vi "Destroy.vi"(8 "error in (no error)":errorcluster, 11 "CIFTag in":refnum<class "CIF_CIPC_Chn.lvclass">) -> (0 "error out":errorcluster, 3 "CIFTag out":refnum<class "CIF_CIPC_Chn.lvclass">)   [LabVIEW 2021, in "CIF_CIPC_Chn.lvclass"]
uses:
  CIF_CIPC_Chn.lvclass
  C:/Program Files/National Instruments/LabVIEW 2021/vi.lib/CIF Foundation/CIF Channels Core/CIFChannels/CIFChannels.lvclass
  <vilib>/CIF Foundation/CIF Channels Core/ChannelCommon/typedef/Channel State.ctl
  Typedef/Buffer Configuration Data.ctl
  <vilib>/CIF Foundation/CIF CIPC/TypeDefs/Backpressure References.ctl
  <vilib>/CIF Foundation/CIF CIPC/TypeDefs/Backpressure Names.ctl
  <vilib>/CIF Foundation/CIF Channels Core/CIFChannels/CIFChannels.lvclass/CIFChannels.ctl
  CIF_CIPC_Chn.lvclass/CIF_CIPC_Chn.ctl
  <vilib>/CIF Foundation/CIF Channels Core/CIFChannels/Accessors/Read Direction.vi
  <vilib>/CIF Foundation/CIF Channels Core/CIFChannels/Accessors/Read FIFO Backpressure.vi
  Accessors/Read Buffer Configuration.vi
  Accessors/Read CIPC Channel.vi
  Accessors/Write Buffer Configuration.vi
  Accessors/Write CIPC Channel.vi
  <vilib>/CIF Foundation/CIF Channels Core/CIFChannels/Accessors/Write Subscriber Count.vi
  <vilib>/CIF Foundation/CIF Channels Core/CIFChannels/Accessors/Write Channel State.vi
  <vilib>/CIF Foundation/CIF CIPC/CIF_NI_CIPC.lvlib
  <vilib>/CIF Foundation/CIF Channels Core/ChannelCommon/ChannelCommon.lvlib
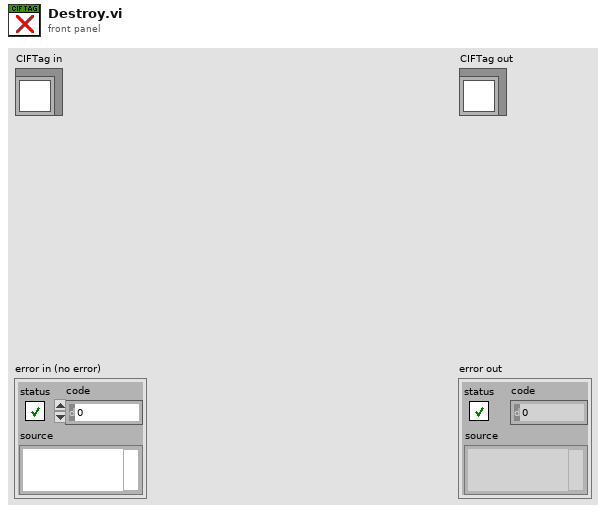
[diagram p1: front panel]
types:
  T1 = typedef "ChannelCommon.lvlib/Channel State.ctl" = enum8{"Creating", "Disconnected", "Connecting", "Connected", "Destroyed"}
  T2 = typedef "CIF_CIPC_Chn.lvclass/Buffer Configuration Data.ctl" = cluster{"Total Size":u32, "Read Size":u32, "Read Offset":u32, "CIPC BP References":T3, "CIPC Backpressure Names":T4, "Override CIPC Name":string, "Encoder Data":string}
  T3 = typedef "CIF_NI_CIPC.lvlib/Backpressure References.ctl" = cluster{"CIPC Reference":u64, "CIPC BP Reference":u64}
  T4 = typedef "CIF_NI_CIPC.lvlib/Backpressure Names.ctl" = cluster{"CIPC Name":string, "CIPC BP Name":string}
  T5 = typedef "ChannelCommon.lvlib/Direction.ctl" = enum8{"Publisher", "Subscriber"}
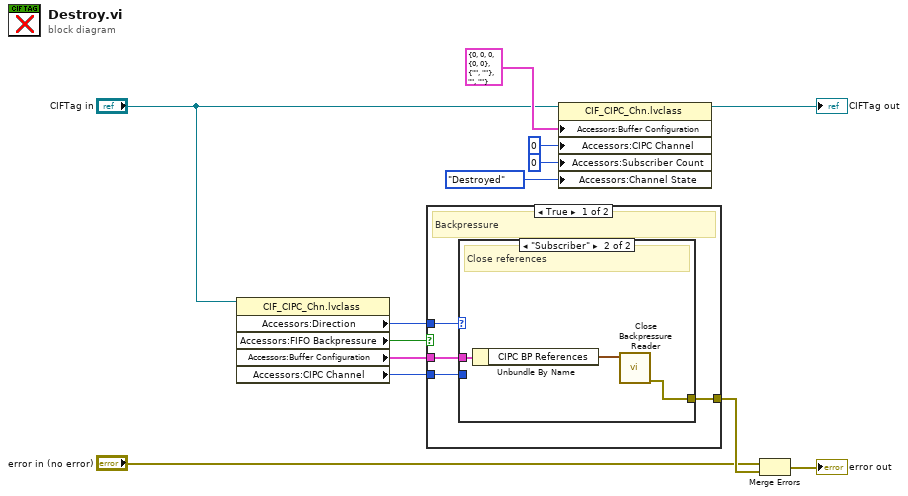
[diagram p0: block diagram]
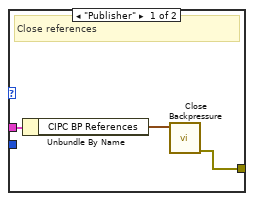
[diagram p2: hidden frame]
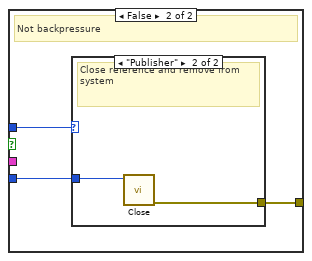
[diagram p3: hidden frame]
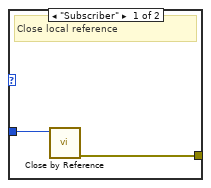
[diagram p4: hidden frame]
diagram:
  n1 = property class="CIF_CIPC_Chn.lvclass"(reference="CIFTag in") -> ("Accessors:Direction"=w13:T5, "Accessors:FIFO Backpressure"=w11:bool, "Accessors:Buffer Configuration"=w10:T2, "Accessors:CIPC Channel"=w12:u64)  [unwired: 1 in, 2 out]
  n2 = case shown="True" w11 {
    tunnel: w13 -> [w17 w26]
    tunnel: w12 -> [w16 w25]
    tunnel: [w14 w24] -> w9
    tunnel: w10 -> [w15 _]
    frame True {
      # "Backpressure"
      n3 = case shown="\"Subscriber\"" w17 {
        tunnel: w16 -> [_ _]
        tunnel: w15 -> [w20 w23]
        tunnel: [w18 w21] -> w14
        frame "Publisher" {
          # "Close references"
          n4 = Unbundle By Name(w20) -> ("CIPC BP References"=w19:T3)
          n5 = call <vilib>:"Close Backpressure.vi"("CIPC BP References in"=w19) -> ("error out"=w18:errorcluster)  [unwired: 10 in]
        }
        frame "Subscriber" {
          # "Close references"
          n6 = Unbundle By Name(w23) -> ("CIPC BP References"=w22:T3)
          n7 = call <vilib>:"Close Backpressure Reader.vi"("CIPC BP References in"=w22) -> ("error out"=w21:errorcluster)  [unwired: 10 in]
        }
      }
    }
    frame False {
      # "Not backpressure"
      n8 = case shown="\"Publisher\"" w26 {
        tunnel: w25 -> [w28 w30]
        tunnel: [w27 w29] -> w24
        frame "Subscriber" {
          # "Close local reference"
          n9 = call <vilib>:"Close by Reference.vi"("CIPC Reference"=w28) -> ("error out"=w27:errorcluster)  [unwired: 10 in]
        }
        frame "Publisher" {
          # "Close reference and remove from system"
          n10 = call <vilib>:"Close.vi"("CIPC Reference"=w30) -> ("error out"=w29:errorcluster)  [unwired: 10 in]
        }
      }
    }
  }
  n11 = property class="CIF_CIPC_Chn.lvclass"(reference="CIFTag in", "Accessors:Buffer Configuration"=T2 {"Total Size"=0, "Read Size"=0, "Read Offset"=0, "CIPC BP References"={"CIPC Reference"=0, "CIPC BP Reference"=0}, "CIPC Backpressure Names"={"CIPC Name"="", "CIPC BP Name"=""}, "Override CIPC Name"="", "Encoder Data"=""} ("Buffer Configuration"), "Accessors:CIPC Channel"=u64 0 ("CIPC Channel"), "Accessors:Subscriber Count"=u32 0 ("Subscriber Count"), "Accessors:Channel State"=Channel_State."Destroyed" ("Channel State")) -> (reference out=→"CIFTag out":refnum<class "CIF_CIPC_Chn.lvclass">)  [unwired: 1 in, 1 out]
  n12 = Merge Errors("error in (no error)", w9) -> (→"error out":errorcluster)
